vi "CheckLastTime.vi"(8 "error in (no error)":errorcluster, 11 "feed GUID":string) -> (0 "error out":errorcluster, 2 "Time Stamp":timestamp)   [LabVIEW 2023, in "GettingStartedWindow.lvlib" / "Feed_link.lvclass"]
uses:
  <resource>/modes/FRC/Classes/Feed_link/Feed_link.lvclass
  <vilib>/Utility/config.llb/NI_LVConfig.lvlib
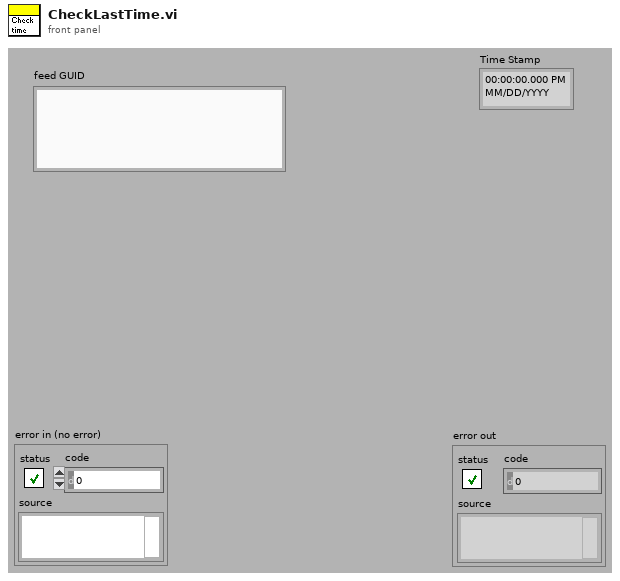
[diagram p1: front panel]
types:
  T1 = typedef "NI_LVConfig.lvlib/Config Data RefNum.ctl" = refnum<k1>
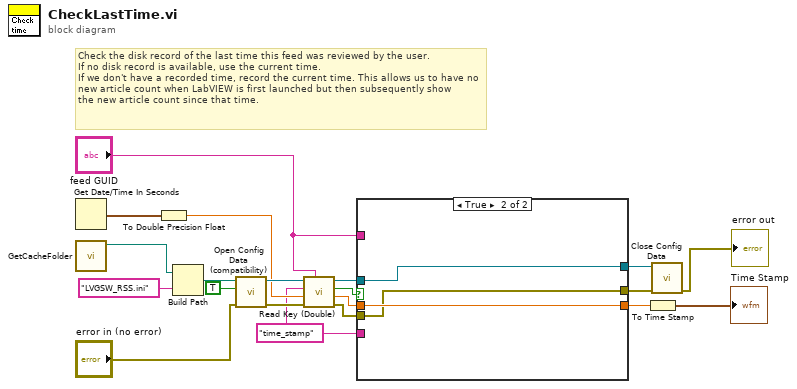
[diagram p0: block diagram]
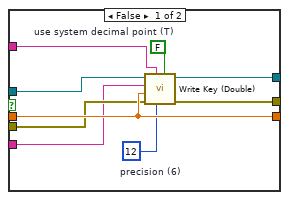
[diagram p2: hidden frame]
diagram:
  w1 = "time_stamp" ("key")
  # "Check the disk record of the last time this feed was reviewed by the user.\nIf no disk record is available, use the current time.\nIf we don't have a recorded time, record the current time. This allows us to have no\nnew article count when LabVIEW is first launched but then subsequently show\nthe new article count since that time."
  n1 = Get Date/Time In Seconds() -> (seconds since 1Jan1904=w15:timestamp)
  n2 = call <resource>:"GetCacheFolder.vi"() -> ("cache folder"=w20:path)  [unwired: 1 in, 10 out]
  n3 = To Double Precision Float(number=w15) -> (double precision float=w12:dbl)
  n4 = Build Path(base path=w20, name or relative path="LVGSW_RSS.ini") -> (appended path=w18:path)
  n5 = call <vilib>:"Open Config Data (compatibility).vi"("error in (no error)"="error in (no error)", "create file if necessary (T)"=TRUE ("create file if necessary? (T)"), "configuration file path"=w18) -> ("error out"=w13:errorcluster, "refnum"=w14:T1)  [unwired: 6 in, 1 out]
  n6 = call <vilib>:"Read Key (Double).vi"("section"="feed GUID", "error in (no error)"=w13, "default value"=w12, "key"=w1, "refnum"=w14) -> ("error out"=w5:errorcluster, "value"=w10:dbl, "found?"=w11:bool, "refnum out"=w8:T1)  [unwired: 3 out]
  n7 = case shown="True" w11 {
    tunnel: w10 -> [w28 w32]
    tunnel: [w28 w32] -> w9
    tunnel: w8 -> [w29 w31]
    tunnel: "feed GUID" -> [w22 _]
    tunnel: [w25 w31] -> w7
    tunnel: w5 -> [w24 w30]
    tunnel: [w23 w30] -> w4
    tunnel: w1 -> [w21 _]
    frame False {
      w26 = i16 12  # precision (6)
      w27 = FALSE  # use system decimal point (T)
      n8 = call <vilib>:"Write Key (Double).vi"("use system decimal point (T)"=w27, "precision (6)"=w26, "section"=w22, "error in (no error)"=w24, "value"=w28, "key"=w21, "refnum"=w29) -> ("error out"=w23:errorcluster, "refnum out"=w25:T1)  [unwired: 1 in, 2 out]
    }
    frame True {
    }
  }
  n9 = To Time Stamp(1:w9) -> (0:→"Time Stamp":timestamp)
  n10 = call <vilib>:"Close Config Data.vi"("error in (no error)"=w4, "refnum"=w7) -> ("error out"=→"error out":errorcluster)  [unwired: 1 in, 8 out]
